vi "Array Test.vi"() -> ()   [LabVIEW 2016]
uses:
  Source/Shared Memory/Controls/file mode.ctl
  Source/Shared Memory/Pointer Operations/In Place Write 1D Array Boolean.vi
  Source/Shared Memory/Pointer Operations/In Place Read 1D Array Boolean.vi
  Source/Shared Memory/Pointer Operations/In Place Write 1D Array DBL.vi
  Source/Shared Memory/Pointer Operations/In Place Read 1D Array DBL.vi
  Source/Shared Memory/Linux RT IPC.Shared Memory.lvlib
  Source/Shared Memory/Classes/Shared Memory/Shared Memory.lvclass
panel:
  out "error out":errorcluster
  in  "stop":bool
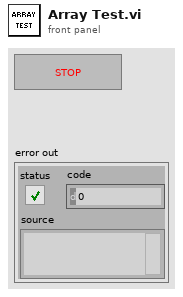
[diagram p1: front panel]
types:
  T1 = typedef "Linux RT IPC.Shared Memory.lvlib/file mode.ctl" = enum16{"open", "create/replace"}
  T2 = typedef "Linux RT IPC.Shared Memory.lvlib/reference.ctl" = refnum<data-value>
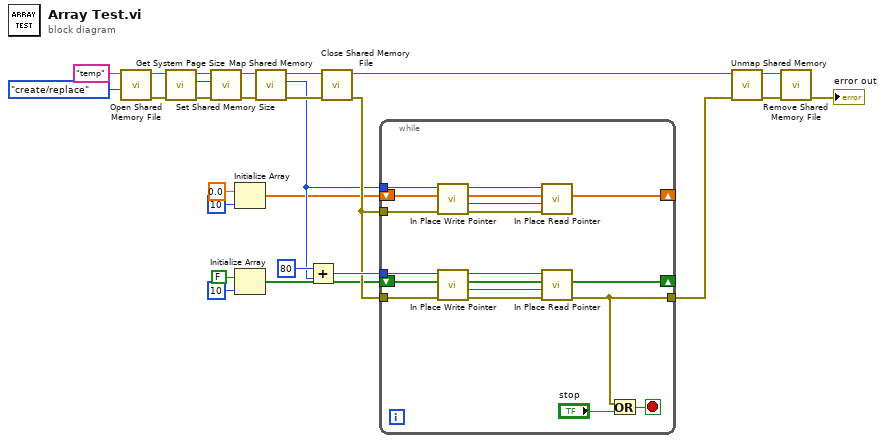
[diagram p0: block diagram]
diagram:
  n1 = call "Open Shared Memory File.vi"("file mode (open)"=file_mode."create/replace" ("file mode (default: open)"), "shared memory name"="temp") -> ("error out"=w19:errorcluster, "shared memory out"=w20:T2)  [unwired: 8 in]
  n2 = call "Get System Page Size.vi"("error in (no error)"=w19, "shared memory in"=w20) -> ("error out"=w14:errorcluster, "page size (bytes)"=w15:u32, "shared memory out"=w18:T2)  [unwired: 7 in]
  n3 = call "Set Shared Memory Size.vi"("error in (no error)"=w14, "size (bytes)"=w15, "shared memory in"=w18) -> ("error out"=w16:errorcluster, "shared memory out"=w17:T2)  [unwired: 7 in]
  n4 = Initialize Array(0.0 ("element"), 10 ("dimension size")) -> (w8:dbl[])
  n5 = Initialize Array(FALSE, 10 ("dimension size")) -> (w7:bool[])
  n6 = call "Map Shared Memory.vi"("error in (no error)"=w16, "shared memory in"=w17) -> ("error out"=w11:errorcluster, "pointer to shared memory"=w9:u64, "shared memory out"=w6:T2)  [unwired: 7 in]
  n7 = Add(x=u64 80 ("y"), y=w9) -> (x+y=w13:u64)
  n8 = call "Close Shared Memory File.vi"("error in (no error)"=w11, "shared memory in"=w6) -> ("error out"=w10:errorcluster, "shared memory out"=w5:T2)  [unwired: 8 in]
  n9 = while {
    shift-right: [w38] -> _
    shift-left: w8 -> [w39]
    shift-right: [w36] -> _
    shift-left: w7 -> [w37]
    tunnel: w9 -> [w33]
    tunnel: w13 -> [w32]
    tunnel: w10 -> [w31]
    tunnel: w10 -> [w30]
    tunnel: [w27] -> w3
    stop <- w28 stop-if-true
    n10 = call-poly "In Place Write Pointer.vi"("error in (no error)"=w31, "values in"=w39, "pointer in"=w33) -> ("error out"=w43:errorcluster, "start index out"=w35:i64, "values out"=w44:dbl[], "pointer out"=w45:u64)  [unwired: 5 in]
    n11 = call-poly "In Place Write Pointer.vi"("error in (no error)"=w30, "values in"=w37, "pointer in"=w32) -> ("error out"=w42:errorcluster, "start index out"=w34:i64, "values out"=w41:bool[], "pointer out"=w40:u64)  [unwired: 5 in]
    n12 = call-poly "In Place Read Pointer.vi"("error in (no error)"=w43, "start index (0)"=w35, "values in"=w44, "pointer in"=w45) -> ("values out"=w38:dbl[])  [unwired: 4 in, 3 out]
    n13 = call-poly "In Place Read Pointer.vi"("error in (no error)"=w42, "start index (0)"=w34, "values in"=w41, "pointer in"=w40) -> ("error out"=w27:errorcluster, "values out"=w36:bool[])  [unwired: 4 in, 2 out]
    n14 = Or(x=w27, y="stop") -> (x .or. y?=w28:bool)
  }
  n15 = call "Unmap Shared Memory.vi"("error in (no error)"=w3, "shared memory in"=w5) -> ("error out"=w2:errorcluster, "shared memory out"=w4:T2)  [unwired: 8 in]
  n16 = call "Remove Shared Memory File.vi"("error in (no error)"=w2, "shared memory in"=w4) -> ("error out"=→"error out":errorcluster)  [unwired: 8 in, 1 out]
